vi "Supervisor_Fault_Procedure.vi"(8 "error in (no error)":errorcluster={"status"=FALSE, "code"=0, "source"="\"\""}, 10 "fault cause":string, 11 "TestDefinition":string) -> (0 "error out":errorcluster={"status"=FALSE, "code"=0, "source"="\"\""}, 2 "status ok":bool, 3 "Procedure outcome":string)   [LabVIEW 2026]
doc: "INTENT: Execute exactly one test-specific fault sequence. LOGIC: Validate permissive safe state, run bounded designated fault sequence, monitor separately; otherwise fallback."
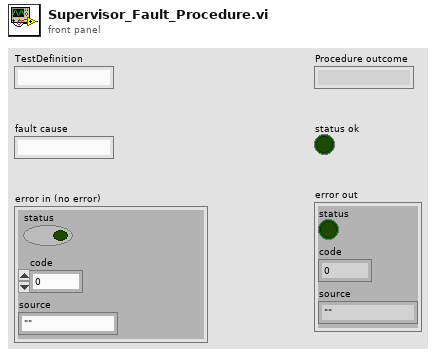
[diagram p1: front panel]
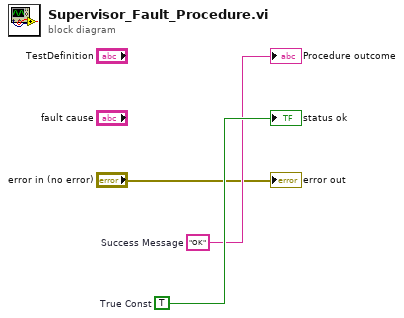
[diagram p0: block diagram]
diagram:
  w3 = TRUE  # True Const
  w2 = "OK"  # Success Message
  "Procedure outcome" <- w2
  "status ok" <- w3
  "error out" <- "error in (no error)"
